vi "piBoardId.vi"(8 "error in (no error)":errorcluster) -> (0 "error out":errorcluster, 1 "mem":i32, 2 "rev":i32, 3 "Model Number":i32, 4 "overVolted":i32, 5 "maker":i32)   [LabVIEW 2020, in "wiringPi.lvlib"]
doc: "<b>_______________________________________________________________</b>\n** Author: Juan José Villacorta\n** LabVIEW wrapper for C library <b> wiringPi </b>,\n** https://github.com/WiringPi/WiringPi\n<b>_______________________________________________________________</b>\n\n*\n * piBoardId:\n * Return the real details of the board we have.\n *\n * This is undocumented and really only intended for the GPIO command.\n * Use at your own risk!\n *\n*/\n\n/*\n * wiringPiSetupGpio:\n * Must be called once at the start of your program execution.\n *\n * GPIO setup: Initialises the system into GPIO Pin mode and uses the\n * memory mapped hardware directly.\n *********************************************************************************\n */"
uses:
  wiringPi.lvlib
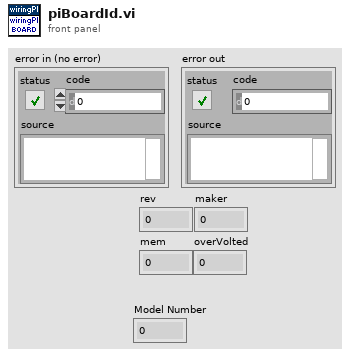
[diagram p1: front panel]
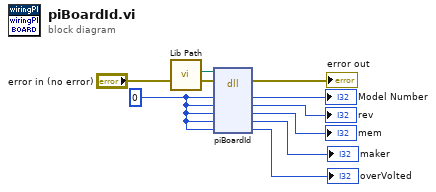
[diagram p0: block diagram]
diagram:
  w6 = 0 ("model")
  n1 = call "Lib Path.vi"() -> ("path out"=w5:path)  [unwired: 11 in]
  n2 = dll-call lib="libLV_wiringPi.so" fn="piBoardId"(path in=w5, error in="error in (no error)", "model"=w6, "rev"=w6, "mem"=w6, "maker"=w6, "overVolted"=w6) -> (error out=→"error out":errorcluster, "model"=→"Model Number":i32, "rev"=→"rev":i32, "mem"=→"mem":i32, "maker"=→"maker":i32, "overVolted"=→"overVolted":i32)  [unwired: 2 in, 1 out]
